vi "VIH HelpGen - Image - Not Found Controls in Conpane Images.vi"(6 "cmd":enum16{"nop", "Init", "Add", "Show"}(ring), 8 "error in":errorcluster, 9 "Conpane Index":i32, 10 "Ctrl Name":string, 11 "VI Name":string) -> (0 "error out":errorcluster)   [LabVIEW 2014]
doc: "::: VI Helpeks :::\nCopyright (c) 2000-2026 Konstantin Shifershteyn. All rights reserved."
panel:
  out "Number":i32
  out "Not Found":string[][](table)
  # "VI Helpeks\nCopyright (c) 2012-2026 Konstantin Shifershteyn"
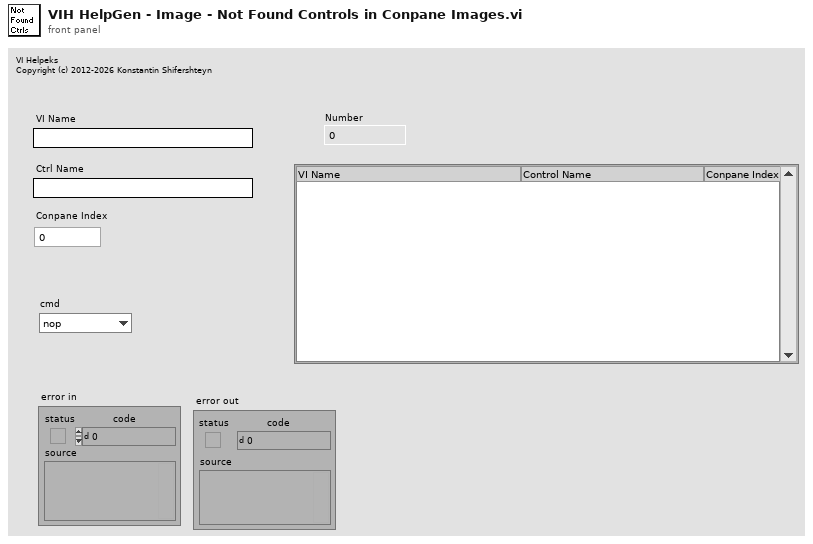
[diagram p1: front panel]
types:
  T1 = cluster{"VI Name":string, "Ctrl Name":string, "Conpane Index":i32}[]
  T2 = cluster{"VI Name":string, "Ctrl Name":string, "Conpane Index":i32}
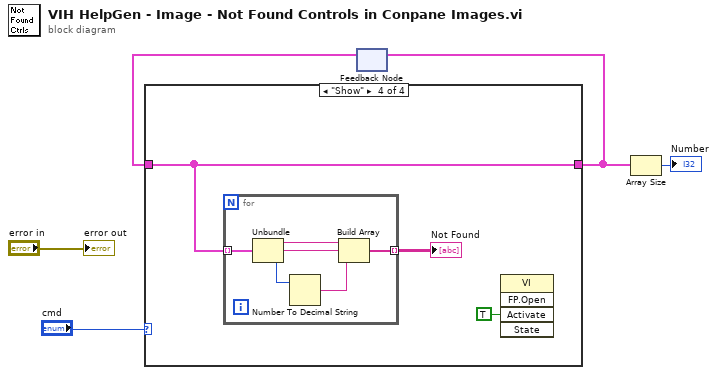
[diagram p0: block diagram]
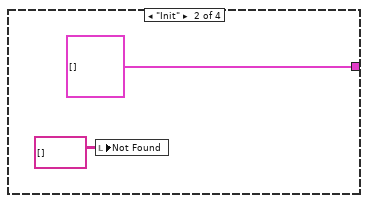
[diagram p3: hidden frame]
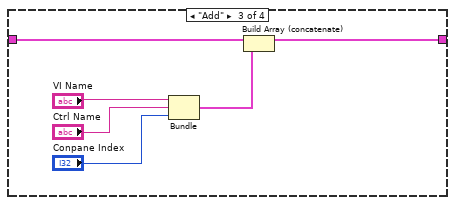
[diagram p4: hidden frame]
diagram:
  n1 = feedback #1() -> (w4:T1)  [unwired: 1 in]
  n2 = case shown="\"Show\"" "cmd" {
    tunnel: w4 -> [w6 _ w10 w17]
    tunnel: [w6 T1 [] w9 w17] -> w3
    frame "nop" {
    }
    frame "Init" {
      n3 = local write "Not Found"(string[][] [] ("Not Found")) -> ()
    }
    frame "Add" {
      n4 = Bundle("VI Name"="VI Name", "Ctrl Name"="Ctrl Name", "Conpane Index"="Conpane Index") -> (w11:T2)  [unwired: 1 in]
      n5 = Build Array (concatenate)(w10, w11) -> (w9:T1)
    }
    frame "Show" {
      n6 = for {
        tunnel: w17 -> [w23] mode=indexing
        tunnel: [w18] -> w16 mode=indexing
        n7 = Unbundle(w23) -> ("VI Name"=w22:string, "Ctrl Name"=w21:string, "Conpane Index"=w20:i32)
        n8 = Number To Decimal String(number=w20) -> (decimal integer string=w19:string)  [unwired: 1 in]
        n9 = Build Array(w22, w21, w19) -> (w18:string[])
      }
      "Not Found" <- w16
      n10 = invoke class="VI" method="FP.Open"("Activate"=TRUE ("Activate?")) -> ()  [unwired: 4 in, 5 out]
    }
  }
  n11 = feedback-in #1(w3) -> ()
  n12 = Array Size(array=w3) -> (size(s)=→"Number":i32)
  "error out" <- "error in"
